vi "Rader graph.vi"(8 "Real B_Comp (NR)":dbl[](array[numeric]), 9 "Real B_Comp (RR)":dbl[](array[numeric]), 10 "XBase_Array_Tag":string[](array[string]), 11 "Theory B_Comp":dbl[](array[numeric])) -> (3 "Radar Plot":picture)   [LabVIEW 2018]
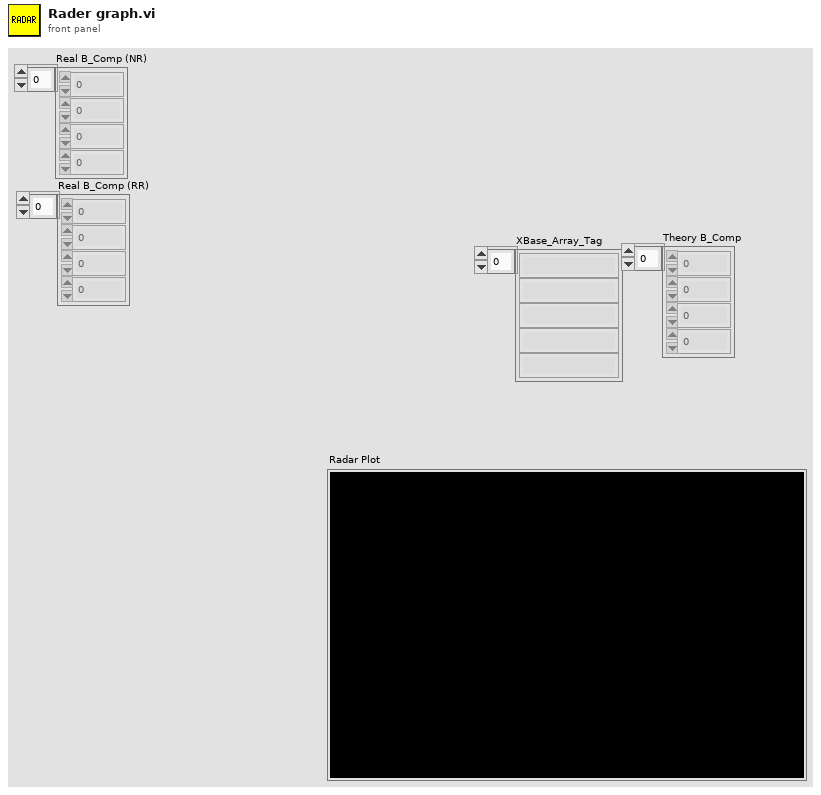
[diagram p1: front panel]
types:
  T1 = cluster{"color (white)":u32, "format and precision":cluster{"format":enum8{"Decimal", "Scientific", "Engineering", "Binary", "Octal", "Hex"}, "precision":u8}, "autoscale? (false)":bool}
  T2 = cluster{"position (none)":enum16{"none", "top", "right", "bottom", "left"}, "text color(white)":u32}
  T3 = typedef "LVBoundsTypeDef.ctl" = cluster{"Width":u32, "Height":u32}
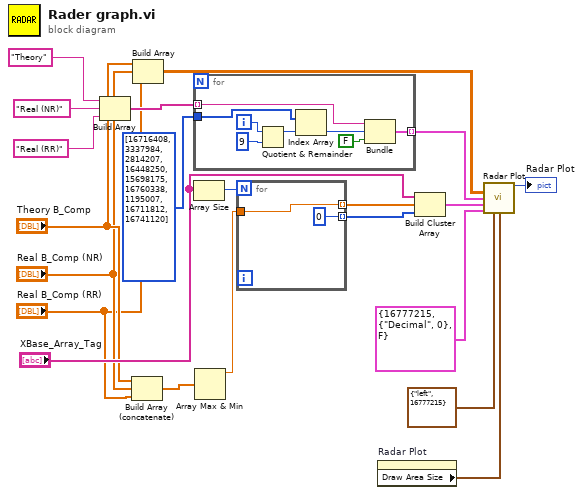
[diagram p0: block diagram]
diagram:
  n1 = Build Array("Theory", "Real (NR)", "Real (RR)") -> (w12:string[])
  n2 = Build Array (concatenate)("Theory B_Comp", "Real B_Comp (NR)", "Real B_Comp (RR)") -> (w3:dbl[])
  n3 = Build Array("Theory B_Comp", "Real B_Comp (NR)", "Real B_Comp (RR)") -> (w10:dbl[][])
  n4 = for {
    tunnel: u32[] [16716408, 3337984, 2814207, 16448250, 15698175, 16760338, 1195007, 16711812, 16741120] -> [w28]
    tunnel: w12 -> [w24] mode=indexing
    tunnel: [w22] -> w20 mode=indexing
    i -> [w29]
    n5 = Quotient & Remainder(x=w29, y=9) -> (x-y*floor(x/y)=w26:i32)  [unwired: 1 out]
    n6 = Index Array(array=w28, index=w26) -> (element=w25:u32)
    n7 = Bundle(w24, w25, FALSE) -> (w22:cluster{string, u32, bool})  [unwired: 1 in]
  }
  n8 = Array Size(array="XBase_Array_Tag") -> (size(s)=w8:i32)
  n9 = Array Max & Min(array=w3) -> (max value=w6:dbl)  [unwired: 3 out]
  n10 = for {
    N: w8 -> [_]
    tunnel: [0] -> w19 mode=indexing
    tunnel: [w30] -> w9 mode=indexing
    tunnel: w6 -> [w30]
  }
  n11 = property on="Radar Plot" class="Pict"() -> ("Draw Area Size"=w16:T3)  [unwired: 2 in, 2 out]
  n12 = Build Cluster Array("XBase_Array_Tag", w9, w19) -> (w18:cluster{string, dbl, i32}[])
  n13 = call <vilib>:"Radar Plot.vi"("data"=w10, "plot info"=w20, "axis info"=w18, "axes info"=T1 {"color (white)"=16777215, "format and precision"={"format"=enum."Decimal", "precision"=0}, "autoscale? (false)"=FALSE}, "legend info"=T2 {"position (none)"=enum."left", "text color(white)"=16777215}, "dimension (w,h)"=w16) -> ("new picture"=→"Radar Plot":picture)  [unwired: 9 in]
